vi "Prcess Data.vi"(8 "error in (no error)":errorcluster, 9 "Running":refnum<vi>, 10 "XY Plot":refnum<vi>, 11 "No Load":refnum<class "No Load Drift.lvclass">) -> (0 "error out":errorcluster, 3 "No Load out":refnum<class "No Load Drift.lvclass">)   [LabVIEW 2025, in "Flow Grind.lvlib" / "No Load Drift.lvclass"]
uses:
  No Load Drift.lvclass
  No Load Drift.lvclass/No Load Drift.ctl
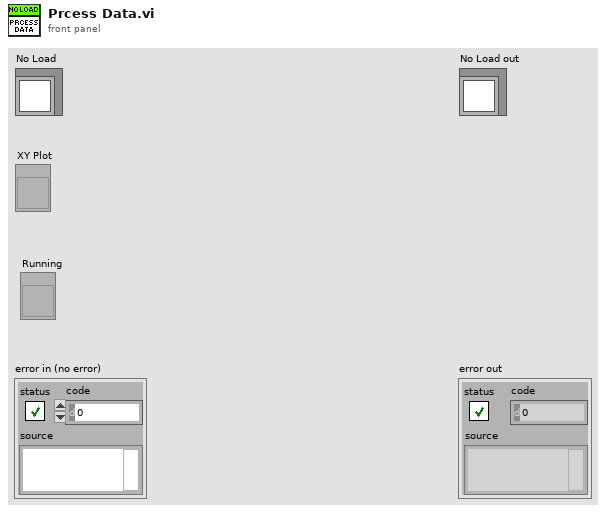
[diagram p1: front panel]
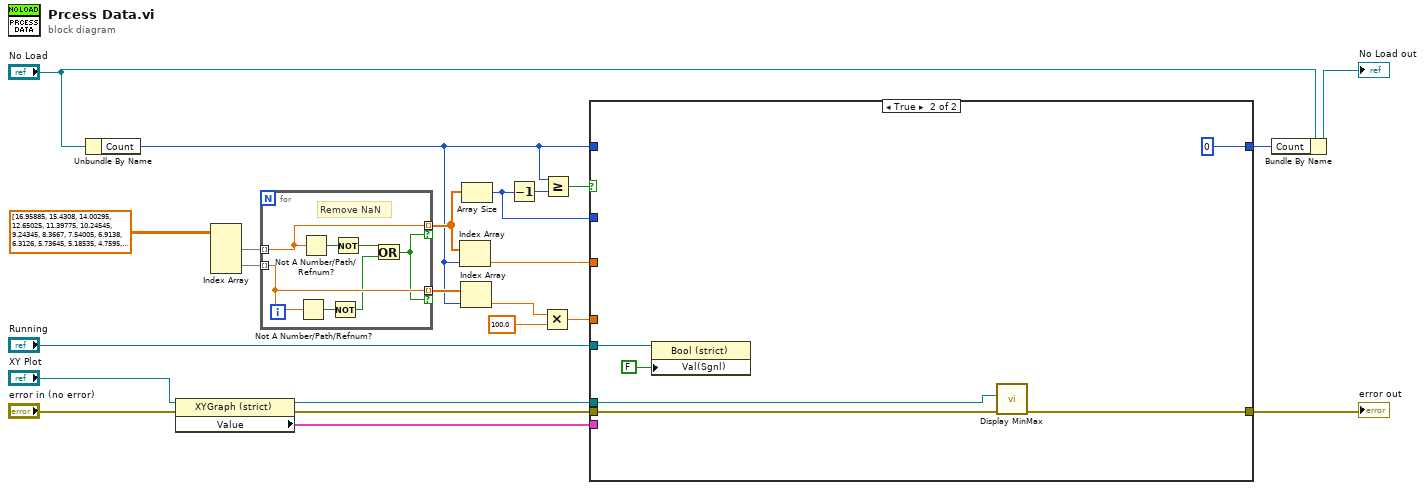
[diagram p0: block diagram]
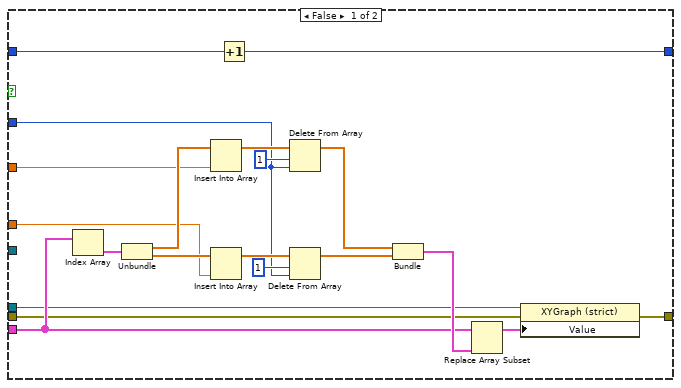
[diagram p2: hidden frame]
diagram:
  n1 = Unbundle By Name("No Load") -> ("Count"=w9:i32)
  n2 = property class="XYGraph (strict)"(reference="XY Plot", error in="error in (no error)") -> (reference out=w10:refnum<vi>, error out=w14:errorcluster, "Value"=w13:cluster{dbl[], dbl[]}[])
  n3 = Index Array(array=dbl[][] [[16.95885, 15.4308, 14.00295, 12.65025, 11.39775, 10.24545, 9.24345, 8.3667, 7.54005, 6.9138, 6.3126, 5.73645, 5.18535, 4.7595, 4.3086, 3.83265, 3.48195, 3.13125, 2.7054, 2.2044, 1.8537, 1.67835, 1.4529, 1.1523, 0.82665, 0.4509, 0.07515, -0.4008, -0.8016, -1.1523, -1.503, -1.82865, -2.2044, -2.47995, -2.7555, -3.08115, -3.507, -4.08315, -4.6593, -5.48595, -6.33765, -7.08915, -7.9659, -8.8176, -9.69435, -10.74645, -11.9238, -13.00095, -14.0781, -14.8797, -15.7314, -16.8837, nan, nan, nan, nan, nan, nan, nan, nan, nan, nan, nan, nan, nan, nan, nan, nan], [-1.6971357, -1.8619372, -2.0524633, -2.293066, -2.5855544, -2.9138894, -3.280457, -3.7018476, -4.190259, -4.6619656, -5.2015096, -5.7941692, -6.423212, -6.9542737, -7.496865, -8.0394363, -8.4269396, -8.643581, -8.4833329, -7.6351319, -6.4527447, -5.5496271, -5.0962598, -5.0705125, -5.5354775, -6.2891462, -6.9633622, -7.5378449, -7.7930267, -7.659218, -7.1905121, -6.6016078, -5.9416192, -5.4885217, -5.0338105, -4.5053239, -3.9360515, -3.4090697, -2.9768439, -2.5476248, -2.1987565, -1.9622422, -1.7476343, -1.556432, -1.3765295, -1.2132742, -1.0540559, -0.9244793, -0.8330689, -0.7598114, -0.6793836, -0.5914539, nan, nan, nan, nan, nan, nan, nan, nan, nan, nan, nan, nan, nan, nan, nan, nan], [0.0, 0.0, 0.0, 0.0, 0.0, 0.0, 0.0, 0.0, 0.0, 0.0, 0.0, 0.0, 0.0, 0.0, 0.0, 0.0, 0.0, 0.0, 0.0, 0.0, 0.0, 0.0, 0.0, 0.0, 0.0, 0.0, 0.0, 0.0, 0.0, 0.0, 0.0, 0.0, 0.0, 0.0, 0.0, 0.0, 0.0, 0.0, 0.0, 0.0, 0.0, 0.0, 0.0, 0.0, 0.0, 0.0, 0.0, 0.0, 0.0, 0.0, 0.0, 0.0, 0.0, 0.0, 0.0, 0.0, 0.0, 0.0, 0.0, 0.0, 0.0, 0.0, 0.0, 0.0, 0.0, 0.0, 0.0, 0.0], [0.0, 0.0, 0.0, 0.0, 0.0, 0.0, 0.0, 0.0, 0.0, 0.0, 0.0, 0.0, 0.0, 0.0, 0.0, 0.0, 0.0, 0.0, 0.0, 0.0, 0.0, 0.0, 0.0, 0.0, 0.0, 0.0, 0.0, 0.0, 0.0, 0.0, 0.0, 0.0, 0.0, 0.0, 0.0, 0.0, 0.0, 0.0, 0.0, 0.0, 0.0, 0.0, 0.0, 0.0, 0.0, 0.0, 0.0, 0.0, 0.0, 0.0, 0.0, 0.0, 0.0, 0.0, 0.0, 0.0, 0.0, 0.0, 0.0, 0.0, 0.0, 0.0, 0.0, 0.0, 0.0, 0.0, 0.0, 0.0]] ("array1")) -> (element #1=w23:dbl[], element #2=w22:dbl[])  [unwired: 4 in]
  n4 = for {
    tunnel: w23 -> [w30] mode=indexing
    tunnel: w22 -> [w27] mode=indexing
    tunnel: [w30] -> w19 mode=indexing if=w24
    tunnel: [w27] -> w21 mode=indexing if=w24
    # "Remove NaN"
    n5 = Not A Number/Path/Refnum?(number/path/refnum=w27) -> (NaN/Path/Refnum?=w28:bool)
    n6 = Not A Number/Path/Refnum?(number/path/refnum=w30) -> (NaN/Path/Refnum?=w29:bool)
    n7 = Not(x=w28) -> (.not. x?=w26:bool)
    n8 = Not(x=w29) -> (.not. x?=w25:bool)
    n9 = Or(x=w25, y=w26) -> (x .or. y?=w24:bool)
  }
  n10 = Index Array(array=w19, index=w9) -> (element=w17:dbl)
  n11 = Index Array(array=w21, index=w9) -> (element=w3:dbl)
  n12 = Array Size(array=w19) -> (size(s)=w8:i32)
  n13 = Decrement(x=w8) -> (x-1=w20:i32)
  n14 = Multiply(x=w3, y=100.0 ("x")) -> (x*y=w2:dbl)
  n15 = Greater Or Equal?(x=w9, y=w20) -> (x >= y?=w18:bool)
  n16 = case shown="True" w18 {
    tunnel: w17 -> [w38 _]
    tunnel: w2 -> [w39 _]
    tunnel: w14 -> [w33 w53]
    tunnel: w13 -> [w40 _]
    tunnel: [w37 0] -> w11
    tunnel: w10 -> [w34 w51]
    tunnel: w9 -> [w36 _]
    tunnel: "Running" -> [_ w55]
    tunnel: w8 -> [w35 _]
    tunnel: [w31 w52] -> w7
    frame False {
      n17 = Index Array(array=w40) -> (element=w49:cluster{dbl[], dbl[]})  [unwired: 1 in]
      n18 = Unbundle(w49) -> (w47:dbl[], w48:dbl[])
      n19 = Insert Into Array(array=w47, new element=w38) -> (w44:dbl[])  [unwired: 1 in]
      n20 = Insert Into Array(array=w48, new element=w39) -> (w45:dbl[])  [unwired: 1 in]
      n21 = Increment(x=w36) -> (x+1=w37:i32)
      n22 = Delete From Array(array=w44, length=1, index=w35) -> (array with subset deleted=w42:dbl[])  [unwired: 1 out]
      n23 = Delete From Array(array=w45, length=1, index=w35) -> (array with subset deleted=w41:dbl[])  [unwired: 1 out]
      n24 = Bundle(w42, w41) -> (w50:cluster{dbl[], dbl[]})  [unwired: 1 in]
      n25 = Replace Array Subset(array=w40, new element=w50) -> (w32:cluster{dbl[], dbl[]}[])  [unwired: 1 in]
      n26 = property class="XYGraph (strict)"(reference=w34, error in=w33, "Value"=w32) -> (error out=w31:errorcluster)  [unwired: 1 out]
    }
    frame True {
      n27 = property class="Bool (strict)"(reference=w55, "Val(Sgnl)"=FALSE ("Value (Signaling)")) -> ()  [unwired: 1 in, 2 out]
      n28 = call "Display MinMax.vi"("error in (no error)"=w53, "Main"=w51) -> ("error out"=w52:errorcluster)  [unwired: 9 in]
    }
  }
  "error out" <- w7
  n29 = Bundle By Name(cluster="No Load", "Count"=w11) -> (→"No Load out":refnum<class "No Load Drift.lvclass">)
